vi "core find or create channel in stream.vi"(9 "tags":map{string, string}(c390), 10 "channel name":string, 11 "stream":refnum<data-value>) -> (0 "error out":errorcluster, 3 "channel":refnum<class "Channel.lvclass">)   [LabVIEW 2020, in "nominal core steps.lvlib"]
doc: "Internal version of the same, using map directly rather than array of tags.\n\nIn the provided stream session, register a channel by name. Tags can only be set on creation and are part of the unique identification of a channel, but are not required.\n\nExamples:\nCall with \"name\", <no tags>; Call with \"name\", <no tags> => one channel\nCall with \"name\", <no tags>; Call with \"name\", tags: [sn: 123] => two channels\nCall with \"name\", tags: [sn: 123]; Call with \"name\", tags: [sn: 321] => two channels\n\n\n\n%docs-exclude%"
uses:
  nominal core steps.lvlib
  <vilib>/Nominal/Nominal IO Client/submodules/nominal-streaming-labview-ffi/lv_src/Channel/Channel.lvclass
  stream session.ctl
  <vilib>/Nominal/Nominal IO Client/submodules/nominal-streaming-labview-ffi/lv_src/Stream/Stream.lvclass
  channel uid.ctl
  <vilib>/Utility/miscctls.llb/LVMapReplaceAction.ctl
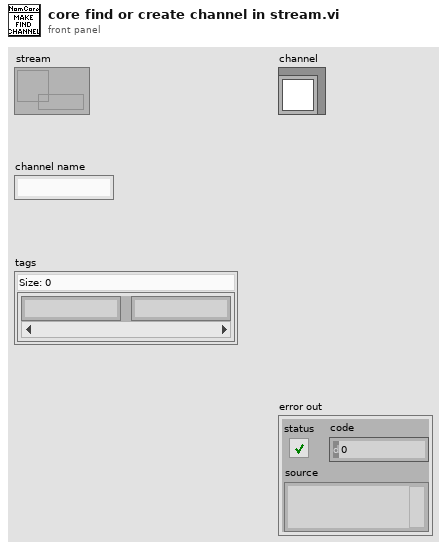
[diagram p1: front panel]
types:
  T1 = typedef "nominal core steps.lvlib/channel uid.ctl" = cluster{"channel name":string, "tags":map{string, string}}
  T2 = typedef "LVMapReplaceAction.ctl" = enum32{"Modify Entry only if found", "Add or Modify Entry", "Delete Entry"}
  T3 = typedef "nominal core steps.lvlib/stream session.ctl" = cluster{"Stream":refnum<class "Stream.lvclass">, "channel cache":map{T1, refnum<class "Channel.lvclass">}}
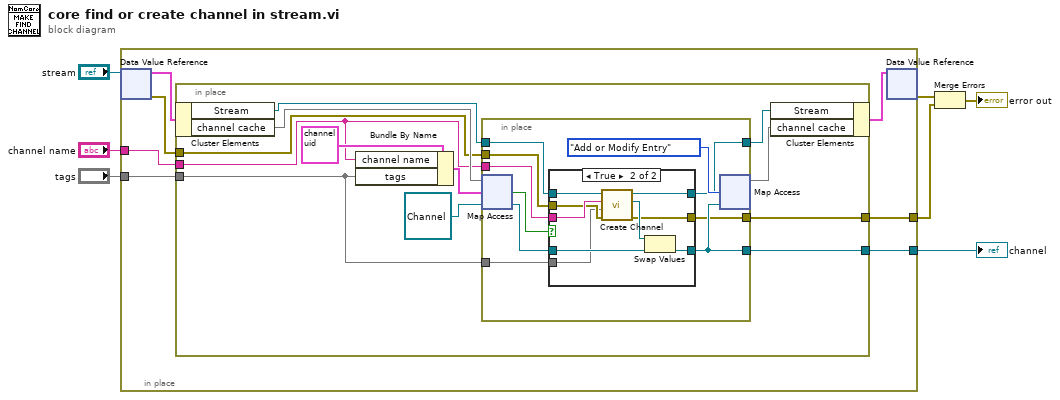
[diagram p0: block diagram]
diagram:
  n1 = in-place {
    in-place-border: "channel name" -> [w12]
    in-place-border: [w11] -> w5
    in-place-border: "tags" -> [w10]
    in-place-border: [w9] -> w6
    n2 = in-place-dvr #1("stream") -> (w14:T3, w8:errorcluster)
    n3 = in-place {
      in-place-border: w12 -> [w17]
      in-place-border: [w21] -> w11
      in-place-border: w10 -> [w15]
      in-place-border: [w20] -> w9
      in-place-border: w8 -> [w19]
      n4 = in-place-cluster #2(w14) -> ("Stream"=w26:refnum<class "Stream.lvclass">, "channel cache"=w23:map{T1, refnum<class "Channel.lvclass">})
      n5 = Bundle By Name(cluster=T1 {"channel name"="", "tags"={}} ("channel unique identifier"), "channel name"=w17, "tags"=w15) -> (w16:T1)
      n6 = in-place {
        in-place-border: w26 -> [w33]
        in-place-border: [w32] -> w25
        in-place-border: w17 -> [w31]
        in-place-border: [w30] -> w21
        in-place-border: [w29] -> w20
        in-place-border: w19 -> [w28]
        in-place-border: w15 -> [w27]
        n7 = in-place-map #3(w23, w16, refnum<class "Channel.lvclass"> refnum ("Channel")) -> (w35:refnum<class "Channel.lvclass">, w36:bool)
        n8 = case shown="True" w36 {
          tunnel: [w39 w46] -> w30
          tunnel: w35 -> [w39 w47]
          tunnel: w33 -> [w38 w45]
          tunnel: [w38 w44] -> w32
          tunnel: w31 -> [_ w43]
          tunnel: [w37 w42] -> w29
          tunnel: w28 -> [w37 w41]
          tunnel: w27 -> [_ w40]
          frame False {
          }
          frame True {
            n9 = call <vilib>:"Create Channel.vi"("error in (no error)"=w41, "Tags"=w40, "Channel Name"=w43, "Nominal Streaming in"=w45) -> ("error out"=w42:errorcluster, "Channel"=w48:refnum<class "Channel.lvclass">, "Nominal Streaming out"=w44:refnum<class "Stream.lvclass">)  [unwired: 5 in]
            n10 = Swap Values(12:w48, 14:w47) -> (3:w46:refnum<class "Channel.lvclass">)  [unwired: 1 in, 1 out]
          }
        }
        n11 = in-place-map #3(w30, LVMapReplaceAction."Add or Modify Entry" ("action")) -> (w22:map{T1, refnum<class "Channel.lvclass">})  [unwired: 2 out]
      }
      n12 = in-place-cluster #2("Stream"=w25, "channel cache"=w22) -> (w13:T3)
    }
    n13 = in-place-dvr #1(w13) -> (w2:errorcluster)  [unwired: 1 out]
  }
  "channel" <- w5
  n14 = Merge Errors(w2, w6) -> (→"error out":errorcluster)
